vi "Calculator.vi"() -> ()   [LabVIEW 2016]
panel:
  out "RESULT":dbl
  out "ZERO DIVISION":bool
  in  "MENU OPTION":T1(ring)
  in  "INPUT 2":dbl
  in  "INPUT 1":dbl
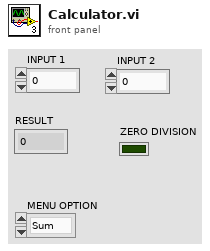
[diagram p1: front panel]
types:
  T1 = enum16{"Sum", "Divide", "Substract", "Multiplpy"}
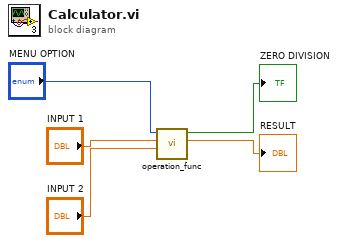
[diagram p0: block diagram]
diagram:
  n1 = call "operation_func.vi"("INPUT in"="INPUT 2", "INPUT 1"="INPUT 1", "MENU OPTION"="MENU OPTION") -> ("Numeric"=→"RESULT":dbl, "Boolean"=→"ZERO DIVISION":bool)  [unwired: 7 in]
